vi "VIH Constant - Help Folder.vi"(11 "append path":path) -> (3 "Help path":path)   [LabVIEW 2014]
doc: "::: VI Helpeks :::\nCopyright (c) 2000-2026 Konstantin Shifershteyn. All rights reserved."
panel:
  # "VI Helpeks\nCopyright (c) 2012-2026 Konstantin Shifershteyn"
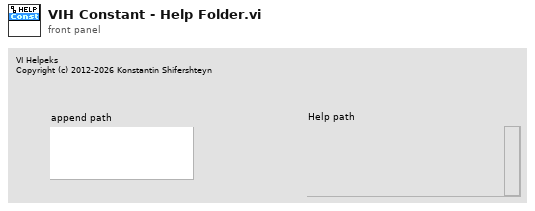
[diagram p1: front panel]
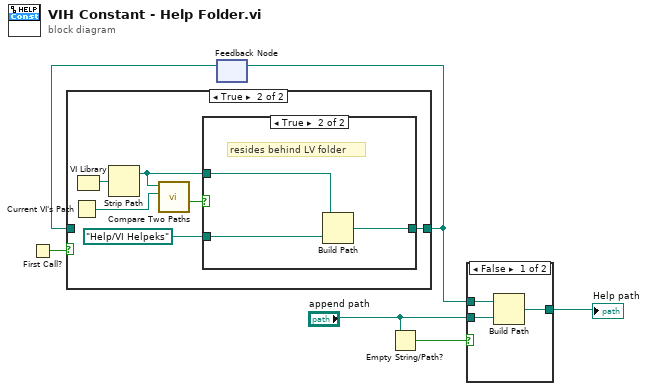
[diagram p0: block diagram]
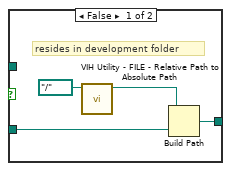
[diagram p3: hidden frame]
diagram:
  n1 = First Call?() -> (First Call?: T/F=w3:bool)
  n2 = feedback #1() -> (w2:path)  [unwired: 1 in]
  n3 = case shown="True" w3 {
    tunnel: [w7 w9] -> w1
    tunnel: w2 -> [w7 _]
    frame False {
    }
    frame True {
      n4 = Current VI's Path() -> (path=w11:path)
      n5 = VI Library() -> (path=w10:path)
      n6 = Strip Path(path=w10) -> (stripped path=w12:path)  [unwired: 1 out]
      n7 = call <vilib>:"Compare Two Paths.vi"("Path 2"=w11, "Path 1"=w12) -> ("Path 2 Relative to Path 1?"=w13:bool)  [unwired: 6 in, 3 out]
      n8 = case shown="True" w13 {
        tunnel: [w17 w20] -> w9
        tunnel: w12 -> [_ w19]
        tunnel: path "Help/VI Helpeks" -> [w14 w18]
        frame False {
          # "resides in development folder"
          n9 = call "VIH Utility - FILE - Relative Path to Absolute Path.vi"("Path"=path "../..") -> ("Path out"=w16:path)  [unwired: 9 in, 1 out]
          n10 = Build Path(base path=w16, name or relative path=w14) -> (appended path=w17:path)
        }
        frame True {
          # "resides behind LV folder"
          n11 = Build Path(base path=w19, name or relative path=w18) -> (appended path=w20:path)
        }
      }
    }
  }
  n12 = feedback-in #1(w1) -> ()
  n13 = Empty String/Path?(string/path="append path") -> (empty?=w4:bool)
  n14 = case shown="False" w4 {
    tunnel: w1 -> [w23 w24]
    tunnel: "append path" -> [w22 _]
    tunnel: [w21 w24] -> w5
    frame False {
      n15 = Build Path(base path=w23, name or relative path=w22) -> (appended path=w21:path)
    }
    frame True {
    }
  }
  "Help path" <- w5
